vi "TestAIO.vi"() -> ()   [LabVIEW 2021]
uses:
  Generic Channel/Channel.lvlib
  Device Channels/Dependencies/AIO-Channel.lvlibp/Channels/AIO-Channel/AIO_Channel_class/AIO_Channel.lvclass
  Device Channels/Dependencies/Channel.lvlibp
  Device Channels/Dependencies/DIO-Channel.lvlibp
  Device Channels/Dependencies/Channel.lvlibp/Channel/Channel_class/Channel.lvclass
  Device Channels/Dependencies/DIO-Channel.lvlibp/Generic Channel/Channel/Channel_class/Channel.lvclass
panel:
  out "Input":dbl
  out "Success":bool
  in  "stop":bool
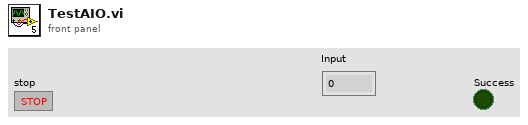
[diagram p1: front panel]
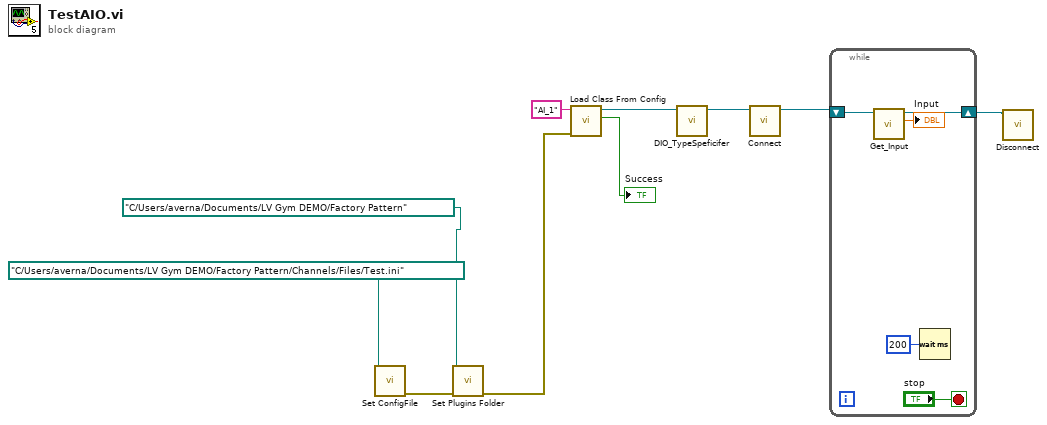
[diagram p0: block diagram]
diagram:
  n1 = call "Set ConfigFile.vi"("Plugins Folder"=path "C:/Users/averna/Documents/LV Gym DEMO/Factory Pattern/Channels/Files/Test.ini" ("Config File")) -> ("error out"=w9:errorcluster)  [unwired: 10 in]
  n2 = call "Set Plugins Folder.vi"("error in (no error)"=w9, "Config File"=path "C:/Users/averna/Documents/LV Gym DEMO/Factory Pattern" ("Plugins Folder")) -> ("error out"=w6:errorcluster)  [unwired: 9 in]
  n3 = call "Load Class From Config.vi"("error in (no error)"=w6, "Name"="AI_1") -> ("Success"=→"Success":bool, "Channel"=w1:refnum<class "Channel.lvclass">)  [unwired: 7 in, 1 out]
  n4 = call "DIO_TypeSpeficifer.vi"("Channel"=w1) -> ("Type_Channel"=w2:refnum<class "DIO_Channel.lvclass">)  [unwired: 9 in, 1 out]
  n5 = call-dynamic "Connect.vi"("object in"=w2) -> ("object out"=w3:refnum<class "AIO_Channel.lvclass">)  [unwired: 8 in, 2 out]
  n6 = while {
    shift-right: [w14] -> w5
    shift-left: w3 -> [w15]
    stop <- "stop" stop-if-true
    n7 = call-dynamic "Get_Input.vi"("object in"=w15) -> ("Input"=→"Input":dbl, "object out"=w14:refnum<class "AIO_Channel.lvclass">)  [unwired: 8 in, 1 out]
    n8 = Wait (ms)(milliseconds to wait=u32 200) -> ()  [unwired: 1 out]
  }
  n9 = call-dynamic "Disconnect.vi"("object in"=w5) -> ()  [unwired: 9 in, 2 out]
